vi "Add Item to Library.vi"(8 "error in":errorcluster, 9 "Item Path":path, 10 "Library":string, 11 "Project Manager in":refnum<class "Project Manager.lvclass">) -> (0 "error out":errorcluster, 3 "Project Manager out":refnum<class "Project Manager.lvclass">)   [LabVIEW 2026, in "Project Manager.lvclass"]
doc: "Add file to a library in the project. The library is specified by name."
uses:
  Project Manager.lvclass
  Project Manager.lvclass/Project Manager.ctl
  <userlib>/_OpenG.lib/file/file.llb/Strip Path Extension - Path__ogtk.vi
  <userlib>/_OpenG.lib/file/file.llb/openg_file.lvlib
  Interfaces/ILogger/ILogger Messages/Log Msg/Log Msg.lvclass
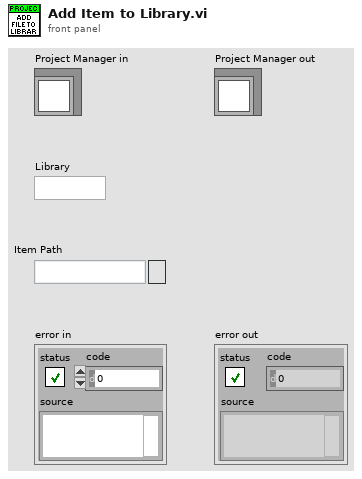
[diagram p1: front panel]
types:
  T1 = typedef "Log Entry--cluster.ctl" = cluster{"Time":timestamp, "Message":string}
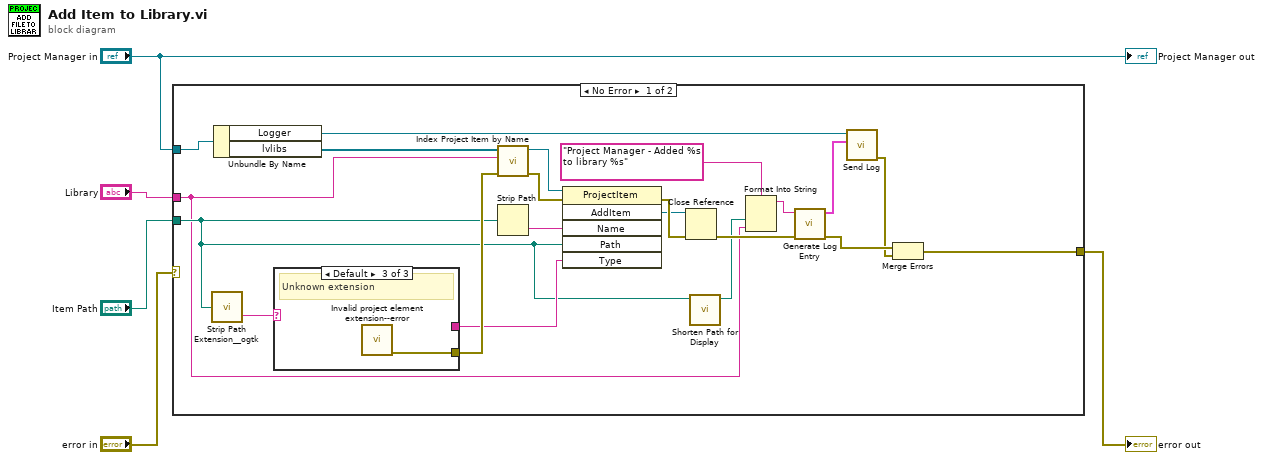
[diagram p0: block diagram]
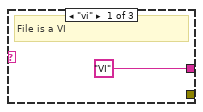
[diagram p2: hidden frame]
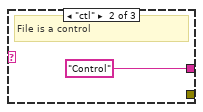
[diagram p3: hidden frame]
diagram:
  n1 = case shown="No Error" "error in" {
    selector: "error in" -> [_ w30]
    tunnel: "Project Manager in" -> [w19 _]
    tunnel: "Item Path" -> [w9 _]
    tunnel: [w21 w30] -> w5
    tunnel: "Library" -> [w7 _]
    frame No Error {
      n2 = call-poly <userlib>:"Strip Path Extension__ogtk.vi"("path"=w9) -> ("extension"=w14:string)  [unwired: 1 out]
      n3 = Unbundle By Name(w19) -> ("Logger"=w12:refnum<class "Message Enqueuer.lvclass">, "lvlibs"=w16:refnum<vi>[])
      n4 = case shown="Default" w14 {
        tunnel: [_ _ w29] -> w24
        tunnel: ["VI" ("Type") "Control" ("Type") _] -> w13
        frame "vi" {
          # "File is a VI"
        }
        frame "ctl" {
          # "File is a control"
        }
        frame Default {
          # "Unknown extension"
          n5 = call "Invalid project element extension--error.vi"() -> ("error out"=w29:errorcluster)  [unwired: 11 in]
        }
      }
      n6 = call "Index Project Item by Name.vi"("error in"=w24, "Name"=w7, "Project Items"=w16) -> ("error out"=w25:errorcluster, "Project Item"=w15:refnum<vi>)  [unwired: 7 in]
      n7 = Strip Path(path=w9) -> (name=w17:string)  [unwired: 1 out]
      n8 = invoke class="ProjectItem" method="AddItem"(reference=w15, error in=w25, "Name"=w17, "Path"=w9, "Type"=w13) -> (error out=w26:errorcluster, "AddItem"=w18:refnum<vi>)  [unwired: 1 in, 4 out]
      n9 = Close Reference(reference=w18, error in (no error)=w26) -> (error out=w23:errorcluster)
      n10 = call "Shorten Path for Display.vi"("Path"=w9) -> ("Shortened Path"=w8:path)  [unwired: 10 in]
      n11 = Format Into String(format string="Project Manager - Added %s to library %s", w8, w7) -> (resulting string=w6:string)  [unwired: 2 in, 1 out]
      n12 = call "Generate Log Entry.vi"("error in"=w23, "Message"=w6) -> ("error out"=w22:errorcluster, "Log Entry"=w11:T1)  [unwired: 8 in]
      n13 = call "Send Log.vi"("Log Entry"=w11, "Message Enqueuer"=w12) -> ("error out"=w20:errorcluster)  [unwired: 8 in, 1 out]
      n14 = Merge Errors(w22, w20) -> (w21:errorcluster)
    }
    frame Error {
      # "Pass error without further action."
    }
  }
  "error out" <- w5
  "Project Manager out" <- "Project Manager in"
